vi "Channel.BuildMenuName.vi"(11 "cluster":T1) -> (3 "NodePath":string)   [LabVIEW 2015, in "Simple Sequence Tools - Shared.lvlib"]
uses:
  Simple Sequence Tools - Shared.lvlib
  Types/Channel.Properties.ctl
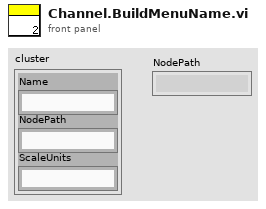
[diagram p1: front panel]
types:
  T1 = typedef "Simple Sequence Tools - Shared.lvlib/Channel.Properties.ctl" = cluster{"Name":string, "NodePath":string, "ScaleUnits":string}
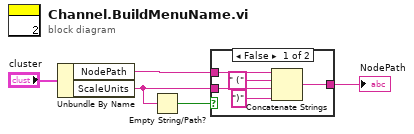
[diagram p0: block diagram]
diagram:
  n1 = Unbundle By Name("cluster") -> ("NodePath"=w2:string, "ScaleUnits"=w4:string)
  n2 = Empty String/Path?(string/path=w4) -> (empty?=w5:bool)
  n3 = case shown="False" w5 {
    tunnel: w2 -> [w8 w11]
    tunnel: [w7 w11] -> w3
    tunnel: w4 -> [w6 _]
    frame False {
      n4 = Concatenate Strings(w8, " (" ("string"), w6, ")" ("string")) -> (w7:string)
    }
    frame True {
    }
  }
  "NodePath" <- w3
